vi "Send TurnTable Complete Event.vi"(8 "error in (no error)":errorcluster caption="에러 입력(에러 없음)", 10 "id":string, 11 "Instrument Manager 입력":refnum<class "Instrument Manager.lvclass">) -> (0 "error out":errorcluster caption="에러 출력", 3 "Instrument Manager 출력":refnum<class "Instrument Manager.lvclass">)   [LabVIEW 2023, in "Instrument Manager.lvclass"]
uses:
  Instrument Manager.lvclass
  TurnTable Complete Event.ctl
  Instrument Manager.lvclass/Instrument Manager.ctl
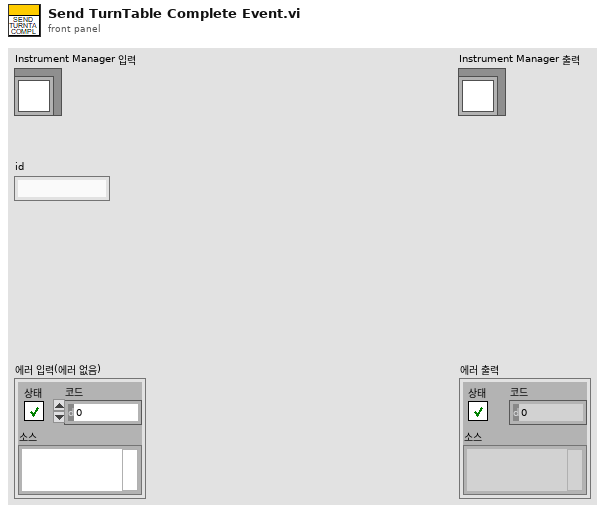
[diagram p1: front panel]
types:
  T1 = typedef "Instrument Manager.lvclass/TurnTable Complete Event.ctl" = cluster{"type":string, "id":string, "target":string, "command":string}
  T2 = cluster{"Reader Q":refnum<queue>, "Writer Q":refnum<queue>}
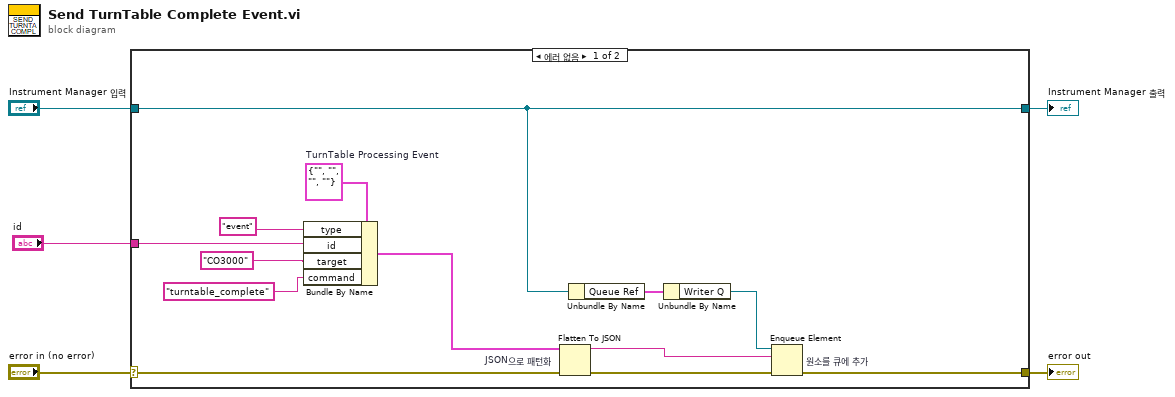
[diagram p0: block diagram]
diagram:
  n1 = case shown="에러 없음" "error in (no error)" {
    selector: "error in (no error)" -> [w9 w19]
    tunnel: [w7 w19] -> w4
    tunnel: [w6 w20] -> w2
    tunnel: "Instrument Manager 입력" -> [w6 w20]
    tunnel: "id" -> [w13 _]
    frame No Error {
      w15 = T1 {"type"="", "id"="", "target"="", "command"=""}  # TurnTable Processing Event
      n2 = Bundle By Name(cluster=w15, "type"="event", "id"=w13, "target"="CO3000", "command"="turntable_complete") -> (w10:T1)
      n3 = Flatten To JSON "JSON으로 패턴화"(anything=w10, error in (no error)=w9) -> (JSON string=w16:string, 11:w8:errorcluster)  [unwired: 1 in]
      n4 = Unbundle By Name(w6) -> ("Queue Ref"=w18:T2)
      n5 = Unbundle By Name(w18) -> ("Writer Q"=w17:refnum<queue>)
      n6 = Enqueue Element "원소를 큐에 추가"(queue=w17, element=w16, error in (no error)=w8) -> (error out=w7:errorcluster)  [unwired: 1 in, 2 out]
    }
    frame Error {
    }
  }
  "error out" <- w4
  "Instrument Manager 출력" <- w2
